vi "DualPump_ExplicitControl_ReverseFlow.vi"() -> ()   [LabVIEW 2025]
uses:
  <vilib>/Utility/error.llb/DialogType.ctl
panel:
  in  "quit":bool
  in  "Tab Control":enum32{"Control Interface", "Info and Help"}(tab)
  out "Pump #2 Sucked Amount (µL)":dbl
  out "Pump #1 Sucked Amount (µL)":dbl
  in  "Pump #2 Start/Stop Button":bool
  in  "Pump #1 COM port":refnum<visa-resource-name>
  in  "Pump #1 flow rate (µL/min)":dbl=2000.0 format="%.3f"
  in  "Pump #2 COM port":refnum<visa-resource-name>
  in  "Pump #2 flow rate (µL/min)":dbl=5000.0 format="%.3f"
  in  "Pump #2 Suck Amount (µL)":dbl=75.0 format="%.3f"
  out "Pump #2 Flowing":bool
  in  "Pump 1 Connect":bool
  in  "Pump 2 Connect":bool
  out "Pump 2 Connected":bool
  out "Pump 1 Connected":bool
  in  "Pump #1 Suck Amount (µL)":dbl=200.0
  in  "Pump #1 Flavor Blast Button":bool
  in  "Pump #1 Start/Stop Button":bool
  out "Pump #1 Flowing":bool
  in  "Pump #2 Flavor Blast Button":bool
  out "Interface Locked":bool
  out "Pump #2 Purging":bool
  in  "Pump #1 Full Purge Button":bool
  in  "Pump #2 Partial Purge Amount (µL)":dbl
  in  "Pump #2 Partial Purge Button":bool
  out "Pump #2 Amount in Syringe (µL)":dbl
  out "Pump #1 Amount in Syringe (µL)":dbl
  in  "Pump #2 syringe volume":dbl(ring)=28.75 items=["5 mL"=11.43, "15 mL"=18.034, "20 mL"=19.79, "50 mL"=28.75]
  in  "Pump #1 syringe volume":dbl(ring)=28.75 items=["5 mL"=11.43, "15 mL"=18.034, "20 mL"=19.79, "50 mL"=28.75, ""=0.0]
  in  "Pump #1 Partial Purge Button":bool
  in  "Pump #2 Full Purge\n Button":bool
  in  "Pump #1 Partial Purge Amount (µL)":dbl
  out "Pump #1 Purging":bool
  # "THIS VI IS FOR DIRECTION-REVERSED FLOW - USE ONLY FOR FILLING SYRINGES AT SET RATES"
  # "1. Set Communication"
  # "Pump #1"
  # "Pump #2"
  # "This program is designed to only control the two New Era Syringe Pumps on-site in the Varro laboratory. It can be generalized for other use by adjusting the hard-coded \"firmware\" variables to match any pump.\n\nFull Purge will empty the syringe completely. Partial Purge will empty the syringe up to the volume injested.\n\nPumps flow continuously when Start is pressed. The pump will suck a specified amount at its flowrate setpoint when Suck It! is pressed.\n\nEmptying and sucking will block the interface, which will be indicated in the upper-right corner."
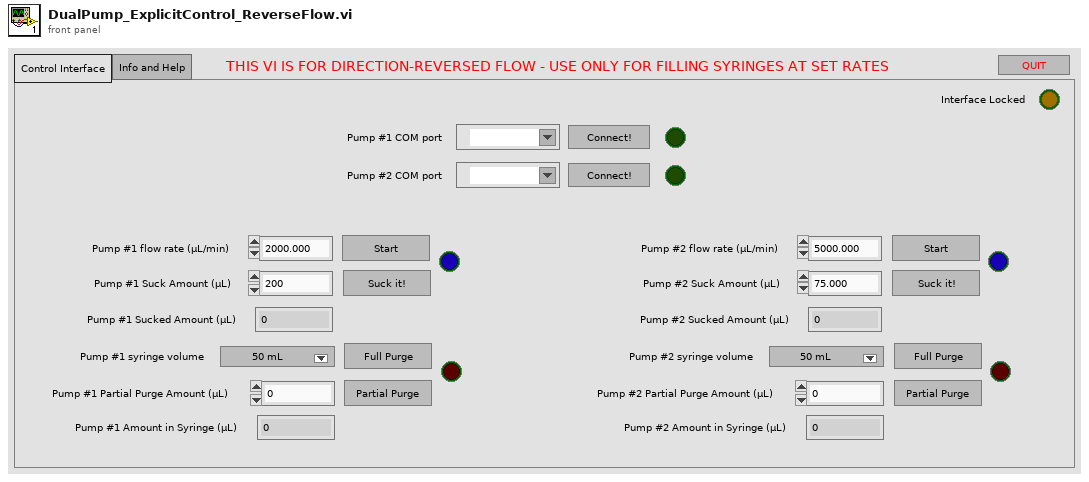
[diagram p1: front panel]
types:
  T1 = cluster{"0=off\n1=on":u16, "Numbers of beeps\n0=continuously":dbl}
  T2 = typedef "DialogType.ctl" = u16
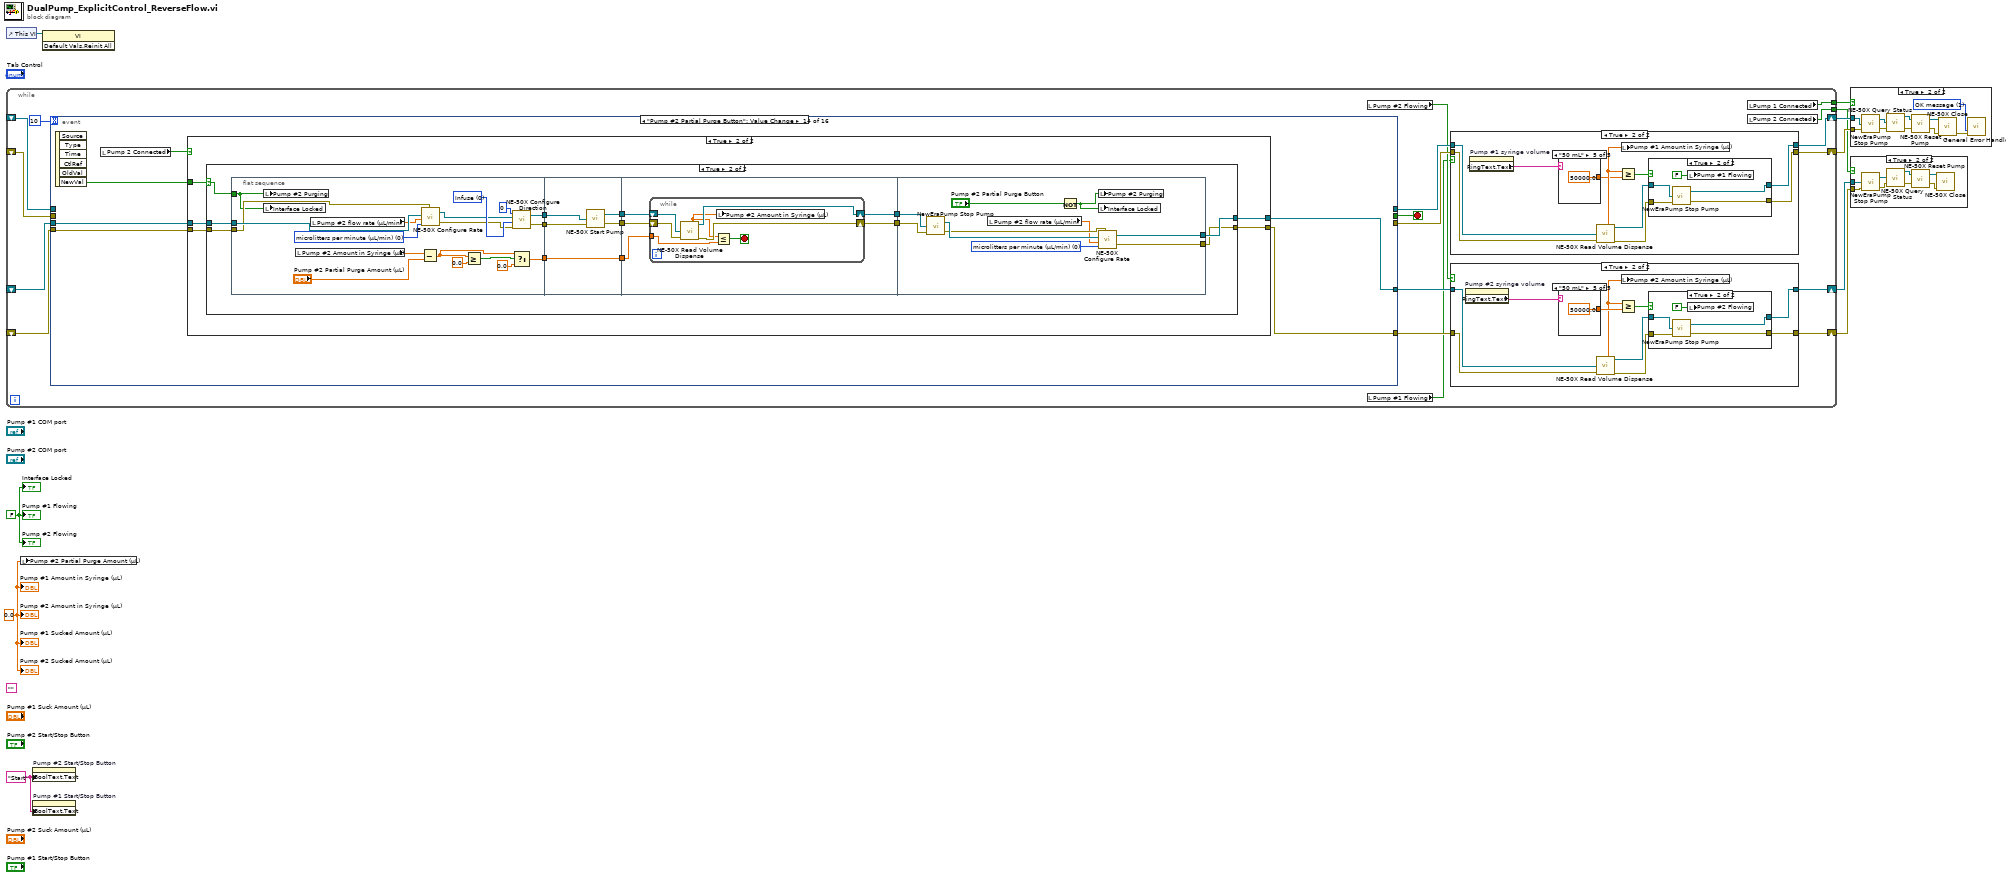
[diagram p0: block diagram]
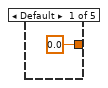
[diagram p6: hidden frame]
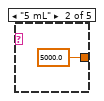
[diagram p7: hidden frame]
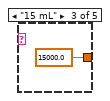
[diagram p8: hidden frame]
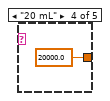
[diagram p9: hidden frame]
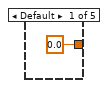
[diagram p12: hidden frame]
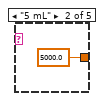
[diagram p13: hidden frame]
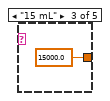
[diagram p14: hidden frame]
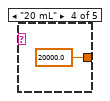
[diagram p15: hidden frame]
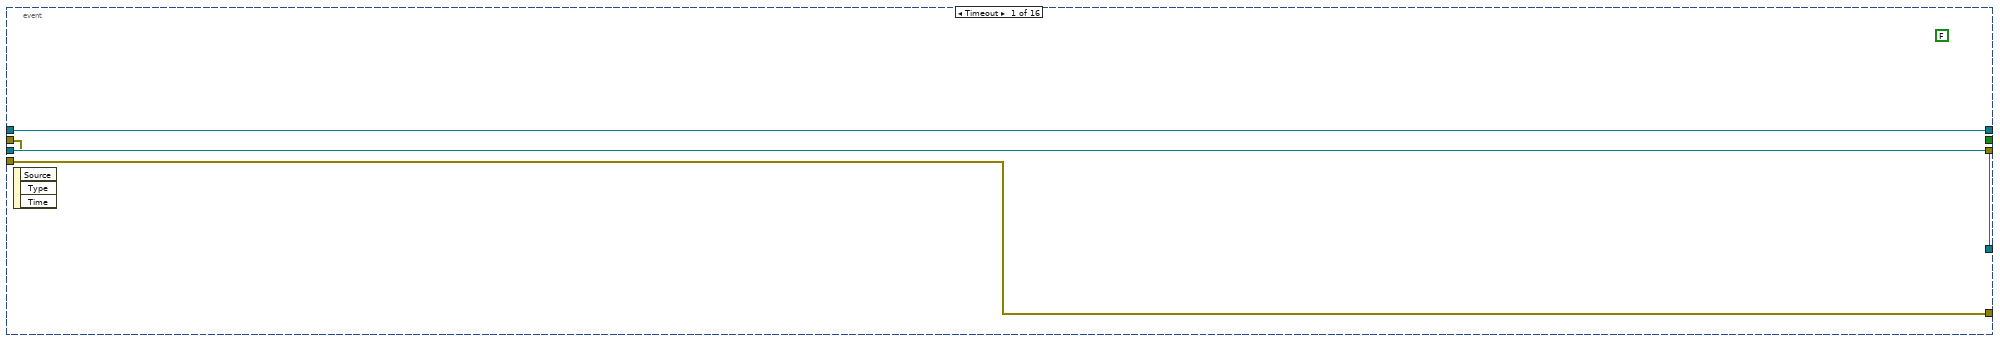
[diagram p16: hidden frame]
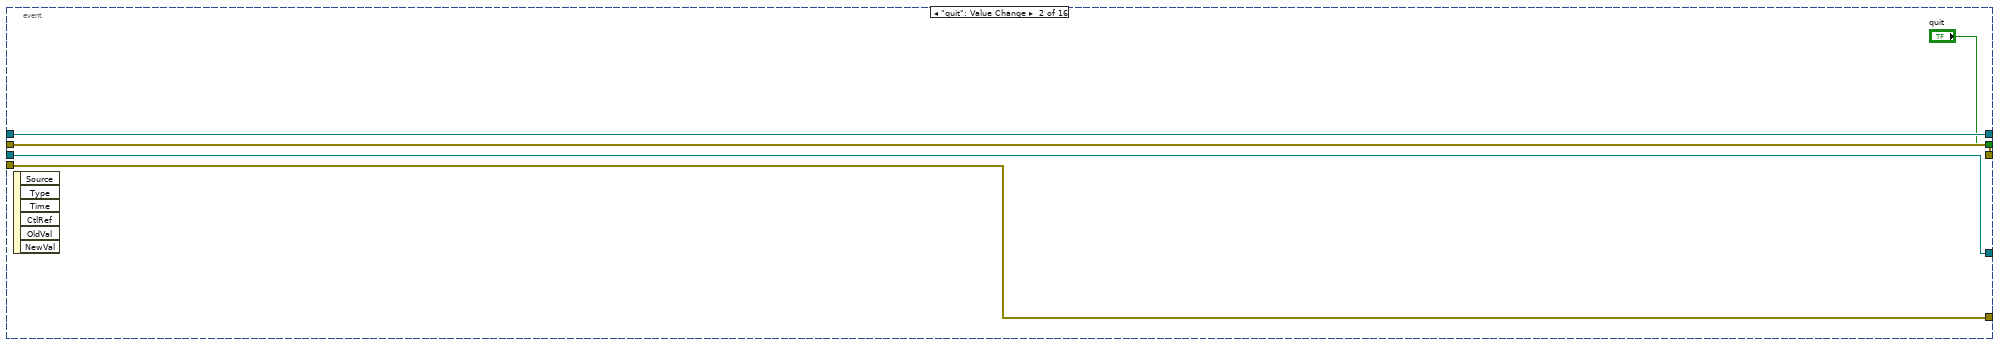
[diagram p17: hidden frame]
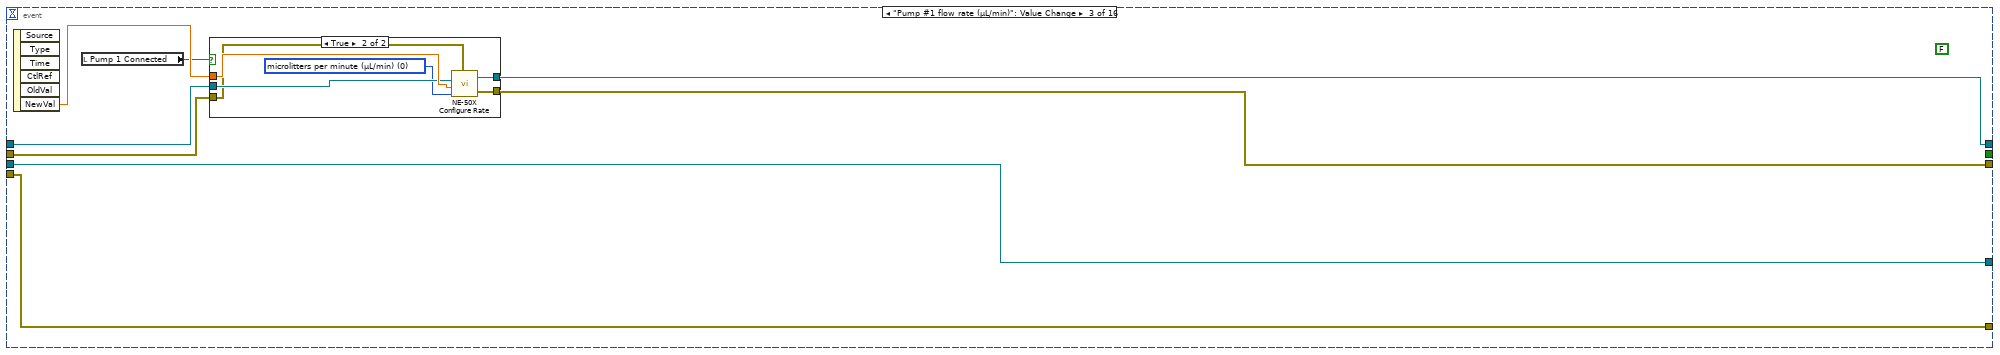
[diagram p18: hidden frame]
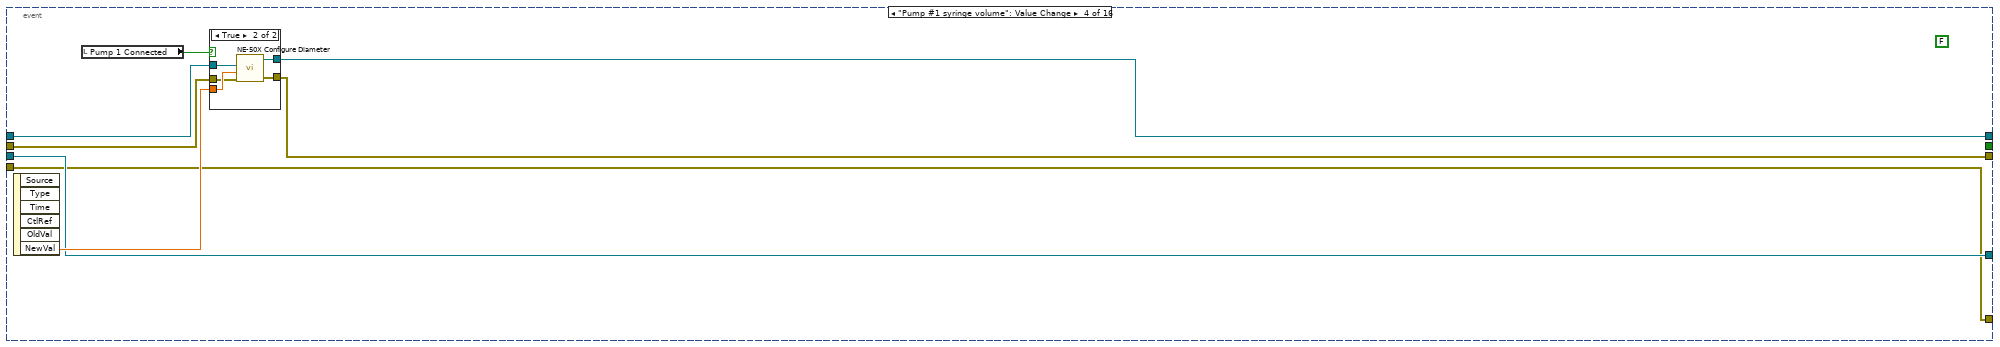
[diagram p20: hidden frame]
diagram:
  w2 = 0.0 ("Pump #1 Flavor Blasted Amount (µL)")
  w1 = FALSE ("0 = Basic")
  w10 = "Start"
  (unwired) ""
  n1 = control-ref of="This VI"() -> (w3:refnum<vi>)
  n2 = while {
    shift-right: [w15] -> w9
    shift-left: _ -> [w28]
    shift-right: [w14] -> w8
    shift-left: _ -> [w27]
    shift-right: [w19] -> w7
    shift-left: _ -> [w25]
    shift-right: [w18] -> w6
    shift-left: _ -> [w26]
    tunnel: [w23] -> w5
    tunnel: [w22] -> w4
    stop <- w11 stop-if-true
    n3 = event shown="[13] \"Pump #2 Partial Purge Button\": Value Change" {
      selector: _ -> [_ _ _ _ _ _ _ _ _ _ _ _ _ _ _ _]
      dyn-events: _ -> [_ _ _ _ _ _ _ _ _ _ _ _ _ _ _ _]
      timeout: 10 -> [_ _ _ _ _ _ _ _ _ _ _ _ _ _ _ _]
      tunnel: w28 -> [w80 w83 w88 w104 w119 w153 w248 w263 w279 w309 w400 _ w476 w555 w629 w706]
      tunnel: w27 -> [w79 w82 w87 w103 w118 w152 w247 w262 w278 w308 w399 _ w475 w554 w628 w705]
      tunnel: w25 -> [w78 w85 w92 w108 w124 w151 w243 w259 w273 w303 _ w439 w481 _ w632 w702]
      tunnel: w26 -> [w77 w84 w91 w107 w122 w150 w242 w258 w272 w301 _ w438 w480 _ w633 w699]
      tunnel: [w80 w83 w88 w104 w119 w147 w246 w261 w275 w307 w400 w441 w476 w553 w629 w701] -> w17
      tunnel: [w79 w82 w87 w103 w118 w148 w245 w260 w274 w306 w399 w440 w475 w552 w628 w700] -> w16
      tunnel: [w78 w85 w90 w106 w123 w146 w243 w259 w273 w304 w403 w439 w478 _ w631 w702] -> w21
      tunnel: [w77 w84 w89 w105 w121 w145 w242 w258 w272 w302 w402 w438 w477 _ w630 w699] -> w20
      tunnel: [_ "quit" _ _ _ _ _ _ _ _ _ _ _ _ _ _] -> w11
      event Timeout {
        (unwired) FALSE ("quit")
        n4 = event-data() -> ()  [unwired: 1 in, 3 out]
      }
      event "quit": Value Change {
        n5 = event-data() -> ()  [unwired: 1 in, 6 out]
      }
      event "Pump #1 flow rate (µL/min)": Value Change {
        (unwired) FALSE ("quit")
        n6 = event-data() -> ("NewVal"=w93:dbl)  [unwired: 1 in, 5 out]
        n7 = local read "Pump 1 Connected"() -> (w86:bool)
        n8 = case shown="True" w86 {
          tunnel: w93 -> [_ w101]
          tunnel: w92 -> [w95 w100]
          tunnel: w91 -> [w94 w99]
          tunnel: [w95 w97] -> w90
          tunnel: [w94 w96] -> w89
          frame False {
          }
          frame True {
            w98 = 0 items=["microlitters per minute (µL/min)", "microlitters per hour (µL/hr)", "milliliters per minute (mL/min)", "milliliters per hour (µL/hr)"] ("Units")
            n9 = call <instrlib>:"NE-50X Configure Rate.vi"("VISA resource name"=w100, "Flow"=w101, "Units"=w98, "error in (no error)"=w99) -> ("VISA resource name out"=w97:refnum<visa-resource-name>, "error out"=w96:errorcluster)  [unwired: 1 in]
          }
        }
      }
      event "Pump #1 syringe volume": Value Change {
        (unwired) FALSE ("quit")
        n10 = event-data() -> ("NewVal"=w109:dbl)  [unwired: 1 in, 5 out]
        n11 = local read "Pump 1 Connected"() -> (w102:bool)
        n12 = case shown="True" w102 {
          tunnel: w109 -> [_ w116]
          tunnel: w108 -> [w110 w115]
          tunnel: w107 -> [w111 w114]
          tunnel: [w110 w113] -> w106
          tunnel: [w111 w112] -> w105
          frame False {
          }
          frame True {
            n13 = call <instrlib>:"NE-50X Configure Diameter.vi"("error in (no error)"=w114, "Diameter (19.58 mm)"=w116, "VISA resource name"=w115) -> ("error out"=w112:errorcluster, "VISA resource name out"=w113:refnum<visa-resource-name>)  [unwired: 1 in, 1 out]
          }
        }
      }
      event "Pump #1 Start/Stop Button": Value Change {
        n14 = event-data() -> ("NewVal"=w120:bool)  [unwired: 1 in, 5 out]
        n15 = local write "Pump #1 Flowing"(w120) -> ()
        n16 = local read "Pump 1 Connected"() -> (w117:bool)
        n17 = case shown="True" w117 {
          tunnel: w124 -> [w126 w131]
          tunnel: [w126 w134] -> w123
          tunnel: w122 -> [w125 w130]
          tunnel: [w125 w133] -> w121
          tunnel: w120 -> [_ w132]
          frame False {
          }
          frame True {
            w129 = u16 1 items=["Infuse", "Withdraw"] ("Direction")
            n18 = call <instrlib>:"NE-50X Configure Direction.vi"("error in (no error)"=w130, "Direction"=w129, "VISA resource name"=w131) -> ("error out"=w127:errorcluster, "VISA resource name out"=w128:refnum<visa-resource-name>)  [unwired: 1 in]
            n19 = case shown="False" w132 {
              tunnel: [w139 w143] -> w134
              tunnel: [w138 w142] -> w133
              tunnel: w128 -> [w136 w141]
              tunnel: w127 -> [w135 w140]
              frame False {
                n20 = call <instrlib>:"NewEraPump Stop Pump.vi"("error in (no error)"=w135, "VISA resource name"=w136) -> ("error out"=w138:errorcluster, "VISA resource name out"=w139:refnum<visa-resource-name>)  [unwired: 1 in]
                n21 = property on="Pump #1 Start/Stop Button" class="Bool"("BoolText.Text"="Start" ("Boolean Text.Text")) -> ()  [unwired: 2 in, 2 out]
              }
              frame True {
                n22 = call <instrlib>:"NE-50X Start Pump.vi"("error in (no error)"=w140, "VISA resource name"=w141) -> ("error out"=w142:errorcluster, "VISA resource name out"=w143:refnum<visa-resource-name>)  [unwired: 1 in]
                n23 = property on="Pump #1 Start/Stop Button" class="Bool"("BoolText.Text"="Stop" ("Boolean Text.Text")) -> ()  [unwired: 2 in, 2 out]
              }
            }
          }
        }
      }
      event "Pump #1 Flavor Blast Button": Value Change {
        (unwired) FALSE ("quit")
        n24 = event-data() -> ("NewVal"=w149:bool)  [unwired: 1 in, 5 out]
        n25 = local read "Pump 1 Connected"() -> (w154:bool)
        n26 = case shown="True" w154 {
          tunnel: w151 -> [w156 w167]
          tunnel: w150 -> [w155 w166]
          tunnel: [w156 w165] -> w146
          tunnel: [w155 w164] -> w145
          tunnel: w149 -> [_ w163]
          tunnel: [w158 w162] -> w147
          tunnel: w153 -> [w158 w161]
          tunnel: [w157 w160] -> w148
          tunnel: w152 -> [w157 w159]
          frame False {
          }
          frame True {
            n27 = case shown="True" w163 {
              selector: w163 -> [_ w174]
              tunnel: w167 -> [w173 w196]
              tunnel: [w171 w190] -> w165
              tunnel: w166 -> [w172 w195]
              tunnel: [w170 w189] -> w164
              tunnel: [w169 w188] -> w162
              tunnel: w161 -> [w169 w185]
              tunnel: [w168 w184] -> w160
              tunnel: w159 -> [w168 w181]
              frame False {
                n28 = call <instrlib>:"NewEraPump Stop Pump.vi"("error in (no error)"=w172, "VISA resource name"=w173) -> ("error out"=w170:errorcluster, "VISA resource name out"=w171:refnum<visa-resource-name>)  [unwired: 1 in]
              }
              frame True {
                n29 = flat-sequence {
                  tunnel: [w200] -> w180
                  tunnel: [w199] -> w179
                  tunnel: [w208] -> w178
                  tunnel: [w207] -> w177
                  tunnel: [w197] -> w175
                  tunnel: w196 -> [w206]
                  tunnel: w195 -> [w205]
                  tunnel: w185 -> [w208]
                  tunnel: w181 -> [w207]
                  tunnel: w174 -> [w198]
                  tunnel: w180 -> [w216]
                  tunnel: w179 -> [w215]
                  tunnel: [w214] -> w194
                  tunnel: [w213] -> w193
                  tunnel: [w212] -> w186
                  tunnel: w178 -> [w212]
                  tunnel: [w211] -> w182
                  tunnel: w177 -> [w211]
                  tunnel: [w210] -> w176
                  tunnel: w175 -> [w210]
                  tunnel: w194 -> [w223]
                  tunnel: w193 -> [w222]
                  tunnel: [w221] -> w192
                  tunnel: [w220] -> w191
                  tunnel: [w219] -> w187
                  tunnel: w186 -> [w219]
                  tunnel: [w218] -> w183
                  tunnel: w182 -> [w218]
                  tunnel: w176 -> [w217]
                  tunnel: w192 -> [w240]
                  tunnel: w191 -> [w239]
                  tunnel: [w238] -> w190
                  tunnel: [w237] -> w189
                  tunnel: [w236] -> w188
                  tunnel: w187 -> [w236]
                  tunnel: [w235] -> w184
                  tunnel: w183 -> [w235]
                  frame #0 {
                    w204 = u16 1 items=["Infuse", "Withdraw"] ("Direction")
                    n30 = local write "Interface Locked"(w198) -> ()
                    n31 = local write "Pump #1 Sucked Amount (µL)"(0.0 ("Pump #1 Flavor Blasted Amount (µL)")) -> ()
                    n32 = call <instrlib>:"NE-50X Configure Direction.vi"("error in (no error)"=w205, "Direction"=w204, "VISA resource name"=w206) -> ("error out"=w202:errorcluster, "VISA resource name out"=w201:refnum<visa-resource-name>)  [unwired: 1 in]
                    n33 = call <instrlib>:"NE-50X Read Volume Dispense.vi"("VISA resource name"=w201, "error in (no error)"=w202) -> ("VISA resource name out"=w200:refnum<visa-resource-name>, "Withdrawn Volume (uL)"=w197:dbl, "error out"=w199:errorcluster)  [unwired: 1 in, 2 out]
                  }
                  frame #1 {
                    n34 = call <instrlib>:"NE-50X Start Pump.vi"("error in (no error)"=w215, "VISA resource name"=w216) -> ("error out"=w213:errorcluster, "VISA resource name out"=w214:refnum<visa-resource-name>)  [unwired: 1 in]
                    n35 = local write "Pump #1 Flowing"(TRUE) -> ()
                  }
                  frame #2 {
                    n36 = while {
                      shift-right: [w230] -> w221
                      shift-left: w223 -> [w233]
                      shift-right: [w229] -> w220
                      shift-left: w222 -> [w232]
                      tunnel: w217 -> [w227]
                      stop <- w231 stop-if-true
                      n37 = call <instrlib>:"NE-50X Read Volume Dispense.vi"("VISA resource name"=w233, "error in (no error)"=w232) -> ("VISA resource name out"=w230:refnum<visa-resource-name>, "Withdrawn Volume (uL)"=w224:dbl, "error out"=w229:errorcluster, "Amount Remaining (uL)"=w225:dbl)  [unwired: 1 in, 1 out]
                      n38 = local read "Pump #1 Suck Amount (µL)"() -> (w228:dbl)
                      n39 = Subtract(x=w224, y=w227) -> (x-y=w226:dbl)
                      n40 = local write "Pump #1 Amount in Syringe (µL)"(w225) -> ()
                      n41 = local write "Pump #1 Sucked Amount (µL)"(w226) -> ()
                      n42 = Greater Or Equal?(x=w226, y=w228) -> (x >= y?=w231:bool)
                    }
                  }
                  frame #3 {
                    w234 = FALSE
                    n43 = call <instrlib>:"NewEraPump Stop Pump.vi"("error in (no error)"=w239, "VISA resource name"=w240) -> ("error out"=w237:errorcluster, "VISA resource name out"=w238:refnum<visa-resource-name>)  [unwired: 1 in]
                    n44 = local write "Pump #1 Flowing"(w234) -> ()
                    n45 = local write "Interface Locked"(w234) -> ()
                  }
                }
              }
            }
          }
        }
      }
      event "Pump #2 flow rate (µL/min)": Value Change {
        (unwired) FALSE ("quit")
        n46 = event-data() -> ("NewVal"=w244:dbl)  [unwired: 1 in, 5 out]
        n47 = local read "Pump 2 Connected"() -> (w241:bool)
        n48 = case shown="True" w241 {
          tunnel: w248 -> [w250 w256]
          tunnel: w247 -> [w249 w255]
          tunnel: [w250 w254] -> w246
          tunnel: [w249 w253] -> w245
          tunnel: w244 -> [_ w252]
          frame False {
          }
          frame True {
            w251 = 0 items=["microlitters per minute (µL/min)", "microlitters per hour (µL/hr)", "milliliters per minute (mL/min)", "milliliters per hour (µL/hr)"] ("Units")
            n49 = call <instrlib>:"NE-50X Configure Rate.vi"("VISA resource name"=w256, "Flow"=w252, "Units"=w251, "error in (no error)"=w255) -> ("VISA resource name out"=w254:refnum<visa-resource-name>, "error out"=w253:errorcluster)  [unwired: 1 in]
          }
        }
      }
      event "Pump #2 syringe volume": Value Change {
        (unwired) FALSE ("quit")
        n50 = event-data() -> ("NewVal"=w264:dbl)  [unwired: 1 in, 5 out]
        n51 = local read "Pump 2 Connected"() -> (w257:bool)
        n52 = case shown="True" w257 {
          tunnel: w264 -> [_ w271]
          tunnel: w263 -> [w265 w270]
          tunnel: w262 -> [w266 w269]
          tunnel: [w265 w268] -> w261
          tunnel: [w266 w267] -> w260
          frame False {
          }
          frame True {
            n53 = call <instrlib>:"NE-50X Configure Diameter.vi"("error in (no error)"=w269, "Diameter (19.58 mm)"=w271, "VISA resource name"=w270) -> ("error out"=w267:errorcluster, "VISA resource name out"=w268:refnum<visa-resource-name>)  [unwired: 1 in, 1 out]
          }
        }
      }
      event "Pump #2 Start/Stop Button": Value Change {
        n54 = event-data() -> ("NewVal"=w276:bool)  [unwired: 1 in, 5 out]
        n55 = local write "Pump #2 Flowing"(w276) -> ()
        n56 = local read "Pump 2 Connected"() -> (w277:bool)
        n57 = case shown="True" w277 {
          tunnel: w279 -> [w281 w286]
          tunnel: [w281 w289] -> w275
          tunnel: w278 -> [w280 w284]
          tunnel: [w280 w288] -> w274
          tunnel: w276 -> [_ w287]
          frame False {
          }
          frame True {
            w282 = u16 1 items=["Infuse", "Withdraw"] ("Direction")
            n58 = call <instrlib>:"NE-50X Configure Direction.vi"("error in (no error)"=w284, "Direction"=w282, "VISA resource name"=w286) -> ("error out"=w283:errorcluster, "VISA resource name out"=w285:refnum<visa-resource-name>)  [unwired: 1 in]
            n59 = case shown="False" w287 {
              tunnel: w285 -> [w294 w298]
              tunnel: [w292 w297] -> w289
              tunnel: w283 -> [w293 w296]
              tunnel: [w291 w295] -> w288
              frame False {
                n60 = call <instrlib>:"NewEraPump Stop Pump.vi"("error in (no error)"=w293, "VISA resource name"=w294) -> ("error out"=w291:errorcluster, "VISA resource name out"=w292:refnum<visa-resource-name>)  [unwired: 1 in]
                n61 = property on="Pump #2 Start/Stop Button" class="Bool"("BoolText.Text"="Start" ("Boolean Text.Text")) -> ()  [unwired: 2 in, 2 out]
              }
              frame True {
                n62 = call <instrlib>:"NE-50X Start Pump.vi"("error in (no error)"=w296, "VISA resource name"=w298) -> ("error out"=w295:errorcluster, "VISA resource name out"=w297:refnum<visa-resource-name>)  [unwired: 1 in]
                n63 = property on="Pump #2 Start/Stop Button" class="Bool"("BoolText.Text"="Stop" ("Boolean Text.Text")) -> ()  [unwired: 2 in, 2 out]
              }
            }
          }
        }
      }
      event "Pump #2 Flavor Blast Button": Value Change {
        (unwired) FALSE ("quit")
        n64 = event-data() -> ("NewVal"=w305:bool)  [unwired: 1 in, 5 out]
        n65 = local read "Pump 2 Connected"() -> (w300:bool)
        n66 = case shown="True" w300 {
          tunnel: w309 -> [w311 w322]
          tunnel: w308 -> [w310 w321]
          tunnel: [w311 w320] -> w307
          tunnel: [w310 w319] -> w306
          tunnel: w305 -> [_ w318]
          tunnel: [w313 w317] -> w304
          tunnel: w303 -> [w313 w316]
          tunnel: [w312 w315] -> w302
          tunnel: w301 -> [w312 w314]
          frame False {
          }
          frame True {
            n67 = case shown="True" w318 {
              selector: w318 -> [_ w330]
              tunnel: w322 -> [w329 w352]
              tunnel: [w327 w346] -> w320
              tunnel: w321 -> [w328 w351]
              tunnel: [w326 w345] -> w319
              tunnel: [w324 w344] -> w317
              tunnel: w316 -> [w324 w341]
              tunnel: [w323 w340] -> w315
              tunnel: w314 -> [w323 w337]
              frame False {
                n68 = property on="Pump #2 Flowing" class="Bool (strict)"("BoolText.Text"="Start" ("Boolean Text.Text")) -> ()  [unwired: 2 in, 2 out]
                n69 = call <instrlib>:"NewEraPump Stop Pump.vi"("error in (no error)"=w328, "VISA resource name"=w329) -> ("error out"=w326:errorcluster, "VISA resource name out"=w327:refnum<visa-resource-name>)  [unwired: 1 in]
              }
              frame True {
                n70 = flat-sequence {
                  tunnel: [w364] -> w336
                  tunnel: [w363] -> w335
                  tunnel: w352 -> [w361]
                  tunnel: w351 -> [w362]
                  tunnel: w341 -> [w364]
                  tunnel: w337 -> [w363]
                  tunnel: [w357] -> w334
                  tunnel: [w356] -> w333
                  tunnel: [w353] -> w331
                  tunnel: w330 -> [w354]
                  tunnel: [w370] -> w350
                  tunnel: [w369] -> w349
                  tunnel: [w368] -> w342
                  tunnel: w336 -> [w368]
                  tunnel: [w367] -> w338
                  tunnel: w335 -> [w367]
                  tunnel: w334 -> [w372]
                  tunnel: w333 -> [w371]
                  tunnel: [w366] -> w332
                  tunnel: w331 -> [w366]
                  tunnel: w350 -> [w379]
                  tunnel: w349 -> [w378]
                  tunnel: [w377] -> w348
                  tunnel: [w376] -> w347
                  tunnel: [w375] -> w343
                  tunnel: w342 -> [w375]
                  tunnel: [w374] -> w339
                  tunnel: w338 -> [w374]
                  tunnel: w332 -> [w373]
                  tunnel: w348 -> [w396]
                  tunnel: w347 -> [w395]
                  tunnel: [w394] -> w346
                  tunnel: [w393] -> w345
                  tunnel: [w392] -> w344
                  tunnel: w343 -> [w392]
                  tunnel: [w391] -> w340
                  tunnel: w339 -> [w391]
                  frame #0 {
                    w360 = u16 1 items=["Infuse", "Withdraw"] ("Direction")
                    n71 = local write "Interface Locked"(w354) -> ()
                    n72 = local write "Pump #2 Sucked Amount (µL)"(0.0 ("Pump #2 Flavor Blasted Amount (µL)")) -> ()
                    n73 = call <instrlib>:"NE-50X Configure Direction.vi"("error in (no error)"=w362, "Direction"=w360, "VISA resource name"=w361) -> ("error out"=w358:errorcluster, "VISA resource name out"=w359:refnum<visa-resource-name>)  [unwired: 1 in]
                    n74 = call <instrlib>:"NE-50X Read Volume Dispense.vi"("VISA resource name"=w359, "error in (no error)"=w358) -> ("VISA resource name out"=w357:refnum<visa-resource-name>, "Withdrawn Volume (uL)"=w353:dbl, "error out"=w356:errorcluster)  [unwired: 1 in, 2 out]
                  }
                  frame #1 {
                    n75 = call <instrlib>:"NE-50X Start Pump.vi"("error in (no error)"=w371, "VISA resource name"=w372) -> ("error out"=w369:errorcluster, "VISA resource name out"=w370:refnum<visa-resource-name>)  [unwired: 1 in]
                    n76 = local write "Pump #2 Flowing"(TRUE) -> ()
                  }
                  frame #2 {
                    n77 = while {
                      shift-right: [w385] -> w377
                      shift-left: w379 -> [w389]
                      shift-right: [w384] -> w376
                      shift-left: w378 -> [w388]
                      tunnel: w373 -> [w383]
                      stop <- w387 stop-if-true
                      n78 = call <instrlib>:"NE-50X Read Volume Dispense.vi"("VISA resource name"=w389, "error in (no error)"=w388) -> ("VISA resource name out"=w385:refnum<visa-resource-name>, "Withdrawn Volume (uL)"=w380:dbl, "error out"=w384:errorcluster, "Amount Remaining (uL)"=w381:dbl)  [unwired: 1 in, 1 out]
                      n79 = local read "Pump #2 Suck Amount (µL)"() -> (w386:dbl)
                      n80 = Subtract(x=w380, y=w383) -> (x-y=w382:dbl)
                      n81 = local write "Pump #2 Amount in Syringe (µL)"(w381) -> ()
                      n82 = local write "Pump #2 Sucked Amount (µL)"(w382) -> ()
                      n83 = Greater Or Equal?(x=w382, y=w386) -> (x >= y?=w387:bool)
                    }
                  }
                  frame #3 {
                    w390 = FALSE
                    n84 = call <instrlib>:"NewEraPump Stop Pump.vi"("error in (no error)"=w395, "VISA resource name"=w396) -> ("error out"=w393:errorcluster, "VISA resource name out"=w394:refnum<visa-resource-name>)  [unwired: 1 in]
                    n85 = local write "Pump #2 Flowing"(w390) -> ()
                    n86 = local write "Interface Locked"(w390) -> ()
                  }
                }
              }
            }
          }
        }
      }
      event "Pump 1 Connect": Value Change {
        w406 = 0 items=["microlitters per minute (µL/min)", "microlitters per hour (µL/hr)", "milliliters per minute (mL/min)", "milliliters per hour (µL/hr)"] ("Units")
        w397 = u16 1 items=["Infuse", "Withdraw"] ("Direction")
        w411 = 0
        w404 = u16 0 items=["Off", "On"] ("0 = Disabled")
        n87 = event-data() -> ()  [unwired: 1 in, 6 out]
        n88 = local read "Pump #1 COM port"() -> (w401:refnum<visa-resource-name>)
        n89 = call <instrlib>:"NE-50X Initialize.vi"("Baud Rate (19200)"=19200, "VISA resource name"=w401) -> ("error out"=w414:errorcluster, "VISA resource name out"=w433:refnum<visa-resource-name>)  [unwired: 1 in]
        n90 = call <instrlib>:"NE-50X Read Firmware Version.vi"("error in (no error)"=w414, "VISA resource name"=w433, "Address (0 if unused)"=w411) -> ("error out"=w415:errorcluster, "Version"=w434:string, "VISA resource name out"=w432:refnum<visa-resource-name>)
        n91 = Equal?(x="NE1000V3.934", y=w434) -> (x = y?=→"Pump 1 Connected":bool)
        n92 = call <instrlib>:"NE-50X Configure Alarms.vi"("error in (no error)"=w415, "Audible Alarms"=FALSE, "VISA resource name"=w432, "Address (0)"=w411) -> ("error out"=w416:errorcluster, "VISA resource name out"=w431:refnum<visa-resource-name>)
        n93 = call <instrlib>:"NE-50X Configure Power Failure Mode.vi"("error in (no error)"=w416, "Power Failure Mode"=w404, "VISA resource name"=w431, "Address (0)"=w411) -> ("error out"=w417:errorcluster, "VISA resource name out"=w430:refnum<visa-resource-name>)
        n94 = call <instrlib>:"NE-50X Configure Safe Mode.vi"("error in (no error)"=w417, "Safe Mode"=FALSE ("0 = Basic"), "VISA resource name"=w430, "Address (0)"=w411) -> ("error out"=w421:errorcluster, "VISA resource name out"=w429:refnum<visa-resource-name>)
        n95 = call <instrlib>:"NE-50X Clear Volumes.vi"("error in (no error)"=w421, "VISA resource name"=w429, "Address (0)"=w411) -> ("error out"=w413:errorcluster, "VISA resource name out"=w428:refnum<visa-resource-name>)
        n96 = call <instrlib>:"NE-50X Configure Diameter.vi"("error in (no error)"=w413, "Diameter (19.58 mm)"="Pump #1 syringe volume", "VISA resource name"=w428, "Address (0)"=w411) -> ("error out"=w422:errorcluster, "VISA resource name out"=w427:refnum<visa-resource-name>)  [unwired: 1 out]
        n97 = call <instrlib>:"NE-50X Configure Rate.vi"("Address (0)"=w411, "VISA resource name"=w427, "Flow"="Pump #1 flow rate (µL/min)", "Units"=w406, "error in (no error)"=w422) -> ("VISA resource name out"=w426:refnum<visa-resource-name>, "error out"=w420:errorcluster)
        n98 = call <instrlib>:"NE-50X Configure Volume.vi"("error in (no error)"=w420, "Volume"=0.0, "VISA resource name"=w426, "Address (0)"=w411) -> ("error out"=w419:errorcluster, "VISA resource name out"=w425:refnum<visa-resource-name>)
        n99 = call <instrlib>:"NE-50X Configure Direction.vi"("error in (no error)"=w419, "Direction"=w397, "VISA resource name"=w425, "Address (0)"=w411) -> ("error out"=w418:errorcluster, "VISA resource name out"=w424:refnum<visa-resource-name>)
        n100 = call <instrlib>:"NE-50X Buzzer.vi"("error in (no error)"=w418, "Buzzer"=T1 {"0=off\n1=on"=0, "Numbers of beeps\n0=continuously"=1.0}, "VISA resource name"=w424, "Address (0)"=w411) -> ("error out"=w402:errorcluster, "VISA resource name out"=w403:refnum<visa-resource-name>)
      }
      event "Pump 2 Connect": Value Change {
        (unwired) FALSE ("quit")
        w448 = 0
        w446 = 0 items=["microlitters per minute (µL/min)", "microlitters per hour (µL/hr)", "milliliters per minute (mL/min)", "milliliters per hour (µL/hr)"] ("Units")
        w436 = u16 1 items=["Infuse", "Withdraw"] ("Direction")
        w444 = u16 0 items=["Off", "On"] ("0 = Disabled")
        n101 = event-data() -> ()  [unwired: 1 in, 6 out]
        n102 = local read "Pump #2 COM port"() -> (w451:refnum<visa-resource-name>)
        n103 = call <instrlib>:"NE-50X Initialize.vi"("Baud Rate (19200)"=19200, "VISA resource name"=w451) -> ("error out"=w453:errorcluster, "VISA resource name out"=w472:refnum<visa-resource-name>)  [unwired: 1 in]
        n104 = call <instrlib>:"NE-50X Read Firmware Version.vi"("error in (no error)"=w453, "VISA resource name"=w472, "Address (0 if unused)"=w448) -> ("error out"=w454:errorcluster, "Version"=w473:string, "VISA resource name out"=w471:refnum<visa-resource-name>)
        n105 = Equal?(x="NE1010V3.934", y=w473) -> (x = y?=→"Pump 2 Connected":bool)
        n106 = call <instrlib>:"NE-50X Configure Alarms.vi"("error in (no error)"=w454, "Audible Alarms"=FALSE, "VISA resource name"=w471, "Address (0)"=w448) -> ("error out"=w455:errorcluster, "VISA resource name out"=w470:refnum<visa-resource-name>)
        n107 = call <instrlib>:"NE-50X Configure Power Failure Mode.vi"("error in (no error)"=w455, "Power Failure Mode"=w444, "VISA resource name"=w470, "Address (0)"=w448) -> ("error out"=w456:errorcluster, "VISA resource name out"=w469:refnum<visa-resource-name>)
        n108 = call <instrlib>:"NE-50X Configure Safe Mode.vi"("error in (no error)"=w456, "Safe Mode"=FALSE ("0 = Basic"), "VISA resource name"=w469, "Address (0)"=w448) -> ("error out"=w460:errorcluster, "VISA resource name out"=w468:refnum<visa-resource-name>)
        n109 = call <instrlib>:"NE-50X Clear Volumes.vi"("error in (no error)"=w460, "VISA resource name"=w468, "Address (0)"=w448) -> ("error out"=w452:errorcluster, "VISA resource name out"=w467:refnum<visa-resource-name>)
        n110 = call <instrlib>:"NE-50X Configure Diameter.vi"("error in (no error)"=w452, "Diameter (19.58 mm)"="Pump #2 syringe volume", "VISA resource name"=w467, "Address (0)"=w448) -> ("error out"=w461:errorcluster, "VISA resource name out"=w466:refnum<visa-resource-name>)  [unwired: 1 out]
        n111 = call <instrlib>:"NE-50X Configure Rate.vi"("Address (0)"=w448, "VISA resource name"=w466, "Flow"="Pump #2 flow rate (µL/min)", "Units"=w446, "error in (no error)"=w461) -> ("VISA resource name out"=w465:refnum<visa-resource-name>, "error out"=w459:errorcluster)
        n112 = call <instrlib>:"NE-50X Configure Volume.vi"("error in (no error)"=w459, "Volume"=0.0, "VISA resource name"=w465, "Address (0)"=w448) -> ("error out"=w458:errorcluster, "VISA resource name out"=w464:refnum<visa-resource-name>)
        n113 = call <instrlib>:"NE-50X Configure Direction.vi"("error in (no error)"=w458, "Direction"=w436, "VISA resource name"=w464, "Address (0)"=w448) -> ("error out"=w457:errorcluster, "VISA resource name out"=w463:refnum<visa-resource-name>)
        n114 = call <instrlib>:"NE-50X Buzzer.vi"("error in (no error)"=w457, "Buzzer"=T1 {"0=off\n1=on"=0, "Numbers of beeps\n0=continuously"=1.0}, "VISA resource name"=w463, "Address (0)"=w448) -> ("error out"=w440:errorcluster, "VISA resource name out"=w441:refnum<visa-resource-name>)
      }
      event "Pump #1 Partial Purge Button": Value Change {
        n115 = event-data() -> ("NewVal"=w479:bool)  [unwired: 1 in, 5 out]
        n116 = local read "Pump 1 Connected"() -> (w482:bool)
        n117 = case shown="True" w482 {
          tunnel: [w484 w489] -> w478
          tunnel: [w483 w488] -> w477
          tunnel: w480 -> [w483 w487]
          tunnel: w481 -> [w484 w486]
          tunnel: w479 -> [_ w485]
          frame False {
          }
          frame True {
            n118 = case shown="True" w485 {
              selector: w485 -> [_ w494]
              tunnel: [w493 w502] -> w489
              tunnel: [w492 w501] -> w488
              tunnel: w487 -> [w490 w498]
              tunnel: w486 -> [w491 w497]
              frame False {
                n119 = call <instrlib>:"NewEraPump Stop Pump.vi"("error in (no error)"=w490, "VISA resource name"=w491) -> ("error out"=w492:errorcluster, "VISA resource name out"=w493:refnum<visa-resource-name>)  [unwired: 1 in]
              }
              frame True {
                n120 = flat-sequence {
                  tunnel: [w524] -> w500
                  tunnel: [w523] -> w499
                  tunnel: [w514] -> w495
                  tunnel: w497 -> [w520]
                  tunnel: w498 -> [w518]
                  tunnel: w494 -> [w513]
                  tunnel: w500 -> [w529]
                  tunnel: w499 -> [w528]
                  tunnel: [w527] -> w506
                  tunnel: [w526] -> w505
                  tunnel: [w525] -> w496
                  tunnel: w495 -> [w525]
                  tunnel: w506 -> [w534]
                  tunnel: w505 -> [w533]
                  tunnel: [w532] -> w504
                  tunnel: [w531] -> w503
                  tunnel: w496 -> [w530]
                  tunnel: w504 -> [w548]
                  tunnel: w503 -> [w547]
                  tunnel: [w549] -> w502
                  tunnel: [w551] -> w501
                  frame #0 {
                    w516 = 0 items=["microlitters per minute (µL/min)", "microlitters per hour (µL/hr)", "milliliters per minute (mL/min)", "milliliters per hour (µL/hr)"] ("Units")
                    w522 = u16 0 items=["Infuse", "Withdraw"] ("Direction")
                    n121 = local write "Pump #1 Purging"(w513) -> ()
                    n122 = local write "Interface Locked"(w513) -> ()
                    n123 = local read "Pump #1 Amount in Syringe (µL)"() -> (w510:dbl)
                    n124 = local read "Pump #1 flow rate (µL/min)"() -> (w512:dbl)
                    n125 = Subtract(x=w510, y="Pump #1 Partial Purge Amount (µL)") -> (x-y=w507:dbl)
                    n126 = call <instrlib>:"NE-50X Configure Rate.vi"("VISA resource name"=w520, "Flow"=w512, "Units"=w516, "error in (no error)"=w518) -> ("VISA resource name out"=w519:refnum<visa-resource-name>, "error out"=w517:errorcluster)  [unwired: 1 in]
                    n127 = Greater Or Equal?(x=w507, y=0.0) -> (x >= y?=w515:bool)
                    n128 = call <instrlib>:"NE-50X Configure Direction.vi"("error in (no error)"=w517, "Direction"=w522, "VISA resource name"=w519, "Address (0)"=0) -> ("error out"=w523:errorcluster, "VISA resource name out"=w524:refnum<visa-resource-name>)
                    n129 = Select(t=w507, s=w515, f=0.0) -> (s? t:f=w514:dbl)
                  }
                  frame #1 {
                    n130 = call <instrlib>:"NE-50X Start Pump.vi"("error in (no error)"=w528, "VISA resource name"=w529) -> ("error out"=w526:errorcluster, "VISA resource name out"=w527:refnum<visa-resource-name>)  [unwired: 1 in]
                  }
                  frame #2 {
                    n131 = while {
                      shift-right: [w539] -> w532
                      shift-left: w534 -> [w541]
                      shift-right: [w538] -> w531
                      shift-left: w533 -> [w540]
                      tunnel: w530 -> [w536]
                      stop <- w537 stop-if-true
                      n132 = call <instrlib>:"NE-50X Read Volume Dispense.vi"("VISA resource name"=w541, "error in (no error)"=w540) -> ("VISA resource name out"=w539:refnum<visa-resource-name>, "error out"=w538:errorcluster, "Amount Remaining (uL)"=w535:dbl)  [unwired: 1 in, 2 out]
                      n133 = Less Or Equal?(x=w535, y=w536) -> (x <= y?=w537:bool)
                      n134 = local write "Pump #1 Amount in Syringe (µL)"(w535) -> ()
                    }
                  }
                  frame #3 {
                    w550 = 0 items=["microlitters per minute (µL/min)", "microlitters per hour (µL/hr)", "milliliters per minute (mL/min)", "milliliters per hour (µL/hr)"] ("Units")
                    n135 = call <instrlib>:"NewEraPump Stop Pump.vi"("error in (no error)"=w547, "VISA resource name"=w548) -> ("error out"=w545:errorcluster, "VISA resource name out"=w546:refnum<visa-resource-name>)  [unwired: 1 in]
                    n136 = local read "Pump #1 flow rate (µL/min)"() -> (w544:dbl)
                    n137 = Not(x="Pump #1 Partial Purge Button") -> (.not. x?=w542:bool)
                    n138 = local write "Pump #1 Purging"(w542) -> ()
                    n139 = local write "Interface Locked"(w542) -> ()
                    n140 = call <instrlib>:"NE-50X Configure Rate.vi"("VISA resource name"=w546, "Flow"=w544, "Units"=w550, "error in (no error)"=w545) -> ("VISA resource name out"=w549:refnum<visa-resource-name>, "error out"=w551:errorcluster)  [unwired: 1 in]
                  }
                }
              }
            }
          }
        }
      }
      event "Pump #2 Partial Purge Button": Value Change {
        n141 = event-data() -> ("NewVal"=w556:bool)  [unwired: 1 in, 5 out]
        n142 = local read "Pump 2 Connected"() -> (w557:bool)
        n143 = case shown="True" w557 {
          tunnel: [w559 w564] -> w553
          tunnel: [w558 w563] -> w552
          tunnel: w554 -> [w558 w562]
          tunnel: w555 -> [w559 w561]
          tunnel: w556 -> [_ w560]
          frame False {
          }
          frame True {
            n144 = case shown="True" w560 {
              selector: w560 -> [_ w569]
              tunnel: [w568 w577] -> w564
              tunnel: [w567 w576] -> w563
              tunnel: w562 -> [w565 w573]
              tunnel: w561 -> [w566 w572]
              frame False {
                n145 = call <instrlib>:"NewEraPump Stop Pump.vi"("error in (no error)"=w565, "VISA resource name"=w566) -> ("error out"=w567:errorcluster, "VISA resource name out"=w568:refnum<visa-resource-name>)  [unwired: 1 in]
              }
              frame True {
                n146 = flat-sequence {
                  tunnel: [w599] -> w575
                  tunnel: [w598] -> w574
                  tunnel: [w582] -> w570
                  tunnel: w572 -> [w595]
                  tunnel: w573 -> [w593]
                  tunnel: w569 -> [w590]
                  tunnel: w575 -> [w604]
                  tunnel: w574 -> [w603]
                  tunnel: [w602] -> w581
                  tunnel: [w601] -> w580
                  tunnel: [w600] -> w571
                  tunnel: w570 -> [w600]
                  tunnel: w581 -> [w609]
                  tunnel: w580 -> [w608]
                  tunnel: [w607] -> w579
                  tunnel: [w606] -> w578
                  tunnel: w571 -> [w605]
                  tunnel: w579 -> [w623]
                  tunnel: w578 -> [w622]
                  tunnel: [w624] -> w577
                  tunnel: [w626] -> w576
                  frame #0 {
                    w591 = 0 items=["microlitters per minute (µL/min)", "microlitters per hour (µL/hr)", "milliliters per minute (mL/min)", "milliliters per hour (µL/hr)"] ("Units")
                    w597 = u16 0 items=["Infuse", "Withdraw"] ("Direction")
                    n147 = local write "Pump #2 Purging"(w590) -> ()
                    n148 = local write "Interface Locked"(w590) -> ()
                    n149 = local read "Pump #2 Amount in Syringe (µL)"() -> (w584:dbl)
                    n150 = local read "Pump #2 flow rate (µL/min)"() -> (w589:dbl)
                    n151 = Subtract(x=w584, y="Pump #2 Partial Purge Amount (µL)") -> (x-y=w585:dbl)
                    n152 = call <instrlib>:"NE-50X Configure Rate.vi"("VISA resource name"=w595, "Flow"=w589, "Units"=w591, "error in (no error)"=w593) -> ("VISA resource name out"=w594:refnum<visa-resource-name>, "error out"=w592:errorcluster)  [unwired: 1 in]
                    n153 = Greater Or Equal?(x=w585, y=0.0) -> (x >= y?=w588:bool)
                    n154 = call <instrlib>:"NE-50X Configure Direction.vi"("error in (no error)"=w592, "Direction"=w597, "VISA resource name"=w594, "Address (0)"=0) -> ("error out"=w598:errorcluster, "VISA resource name out"=w599:refnum<visa-resource-name>)
                    n155 = Select(t=w585, s=w588, f=0.0) -> (s? t:f=w582:dbl)
                  }
                  frame #1 {
                    n156 = call <instrlib>:"NE-50X Start Pump.vi"("error in (no error)"=w603, "VISA resource name"=w604) -> ("error out"=w601:errorcluster, "VISA resource name out"=w602:refnum<visa-resource-name>)  [unwired: 1 in]
                  }
                  frame #2 {
                    n157 = while {
                      shift-right: [w614] -> w607
                      shift-left: w609 -> [w616]
                      shift-right: [w613] -> w606
                      shift-left: w608 -> [w615]
                      tunnel: w605 -> [w611]
                      stop <- w612 stop-if-true
                      n158 = call <instrlib>:"NE-50X Read Volume Dispense.vi"("VISA resource name"=w616, "error in (no error)"=w615) -> ("VISA resource name out"=w614:refnum<visa-resource-name>, "error out"=w613:errorcluster, "Amount Remaining (uL)"=w610:dbl)  [unwired: 1 in, 2 out]
                      n159 = Less Or Equal?(x=w610, y=w611) -> (x <= y?=w612:bool)
                      n160 = local write "Pump #2 Amount in Syringe (µL)"(w610) -> ()
                    }
                  }
                  frame #3 {
                    w625 = 0 items=["microlitters per minute (µL/min)", "microlitters per hour (µL/hr)", "milliliters per minute (mL/min)", "milliliters per hour (µL/hr)"] ("Units")
                    n161 = call <instrlib>:"NewEraPump Stop Pump.vi"("error in (no error)"=w622, "VISA resource name"=w623) -> ("error out"=w620:errorcluster, "VISA resource name out"=w621:refnum<visa-resource-name>)  [unwired: 1 in]
                    n162 = local read "Pump #2 flow rate (µL/min)"() -> (w619:dbl)
                    n163 = Not(x="Pump #2 Partial Purge Button") -> (.not. x?=w617:bool)
                    n164 = local write "Pump #2 Purging"(w617) -> ()
                    n165 = local write "Interface Locked"(w617) -> ()
                    n166 = call <instrlib>:"NE-50X Configure Rate.vi"("VISA resource name"=w621, "Flow"=w619, "Units"=w625, "error in (no error)"=w620) -> ("VISA resource name out"=w624:refnum<visa-resource-name>, "error out"=w626:errorcluster)  [unwired: 1 in]
                  }
                }
              }
            }
          }
        }
      }
      event "Pump #1 Full Purge Button": Value Change {
        n167 = event-data() -> ("NewVal"=w627:bool)  [unwired: 1 in, 5 out]
        n168 = local read "Pump 1 Connected"() -> (w634:bool)
        n169 = case shown="True" w634 {
          tunnel: [w636 w641] -> w631
          tunnel: [w635 w640] -> w630
          tunnel: w633 -> [w635 w639]
          tunnel: w632 -> [w636 w638]
          tunnel: w627 -> [_ w637]
          frame False {
          }
          frame True {
            n170 = case shown="True" w637 {
              selector: w637 -> [_ w646]
              tunnel: [w645 w652] -> w641
              tunnel: [w644 w651] -> w640
              tunnel: w639 -> [w642 w648]
              tunnel: w638 -> [w643 w647]
              frame False {
                n171 = call <instrlib>:"NewEraPump Stop Pump.vi"("error in (no error)"=w642, "VISA resource name"=w643) -> ("error out"=w644:errorcluster, "VISA resource name out"=w645:refnum<visa-resource-name>)  [unwired: 1 in]
              }
              frame True {
                n172 = flat-sequence {
                  tunnel: [w668] -> w650
                  tunnel: [w667] -> w649
                  tunnel: w647 -> [w664]
                  tunnel: w648 -> [w662]
                  tunnel: w646 -> [w657]
                  tunnel: w650 -> [w677]
                  tunnel: w649 -> [w676]
                  tunnel: [w675] -> w656
                  tunnel: [w674] -> w655
                  tunnel: w656 -> [w681]
                  tunnel: w655 -> [w680]
                  tunnel: [w679] -> w654
                  tunnel: [w678] -> w653
                  tunnel: w654 -> [w695]
                  tunnel: w653 -> [w693]
                  tunnel: [w696] -> w652
                  tunnel: [w698] -> w651
                  frame #0 {
                    w660 = 2 items=["microlitters per minute (µL/min)", "microlitters per hour (µL/hr)", "milliliters per minute (mL/min)", "milliliters per hour (µL/hr)"] ("Units")
                    w666 = u16 0 items=["Infuse", "Withdraw"] ("Direction")
                    n173 = local write "Interface Locked"(w657) -> ()
                    n174 = property on="Pump #1 syringe volume" class="Ring (strict)"() -> ("RingText.Text"=w659:string)  [unwired: 2 in, 2 out]
                    n175 = case shown="\"50 mL\"" w659 {
                      tunnel: [0.0 ("y") 5.0 ("y") 13.0 ("y") 14.0 ("y") 30.0 ("y")] -> w658
                      frame Default {
                      }
                      frame "5 mL" {
                      }
                      frame "15 mL" {
                      }
                      frame "20 mL" {
                      }
                      frame "50 mL" {
                      }
                    }
                    n176 = call <instrlib>:"NE-50X Configure Rate.vi"("VISA resource name"=w664, "Flow"=w658, "Units"=w660, "error in (no error)"=w662) -> ("VISA resource name out"=w663:refnum<visa-resource-name>, "error out"=w661:errorcluster)  [unwired: 1 in]
                    n177 = call <instrlib>:"NE-50X Configure Direction.vi"("error in (no error)"=w661, "Direction"=w666, "VISA resource name"=w663, "Address (0)"=0) -> ("error out"=w667:errorcluster, "VISA resource name out"=w668:refnum<visa-resource-name>)
                    "Pump #1 Purging" <- w657
                  }
                  frame #1 {
                    n178 = call <instrlib>:"NE-50X Start Pump.vi"("error in (no error)"=w676, "VISA resource name"=w677) -> ("error out"=w674:errorcluster, "VISA resource name out"=w675:refnum<visa-resource-name>)  [unwired: 1 in]
                  }
                  frame #2 {
                    n179 = while {
                      shift-right: [w686] -> w679
                      shift-left: w681 -> [w688]
                      shift-right: [w685] -> w678
                      shift-left: w680 -> [w687]
                      stop <- w682 stop-if-true
                      n180 = call <instrlib>:"NE-50X Read Volume Dispense.vi"("VISA resource name"=w688, "error in (no error)"=w687) -> ("VISA resource name out"=w686:refnum<visa-resource-name>, "error out"=w685:errorcluster, "Amount Remaining (uL)"=w684:dbl)  [unwired: 1 in, 2 out]
                      n181 = local write "Pump #1 Amount in Syringe (µL)"(w684) -> ()
                      n182 = Less Or Equal?(x=w684, y=0.0) -> (x <= y?=w682:bool)
                    }
                  }
                  frame #3 {
                    w697 = 0 items=["microlitters per minute (µL/min)", "microlitters per hour (µL/hr)", "milliliters per minute (mL/min)", "milliliters per hour (µL/hr)"] ("Units")
                    n183 = call <instrlib>:"NewEraPump Stop Pump.vi"("error in (no error)"=w693, "VISA resource name"=w695) -> ("error out"=w692:errorcluster, "VISA resource name out"=w694:refnum<visa-resource-name>)  [unwired: 1 in]
                    n184 = local read "Pump #1 flow rate (µL/min)"() -> (w691:dbl)
                    n185 = Not(x="Pump #1 Full Purge Button") -> (.not. x?=w689:bool)
                    n186 = local write "Pump #1 Purging"(w689) -> ()
                    n187 = local write "Interface Locked"(w689) -> ()
                    n188 = call <instrlib>:"NE-50X Configure Rate.vi"("VISA resource name"=w694, "Flow"=w691, "Units"=w697, "error in (no error)"=w692) -> ("VISA resource name out"=w696:refnum<visa-resource-name>, "error out"=w698:errorcluster)  [unwired: 1 in]
                  }
                }
              }
            }
          }
        }
      }
      event "Pump #2 Full Purge\n Button": Value Change {
        n189 = event-data() -> ("NewVal"=w704:bool)  [unwired: 1 in, 5 out]
        n190 = local read "Pump 2 Connected"() -> (w703:bool)
        n191 = case shown="True" w703 {
          tunnel: [w708 w713] -> w701
          tunnel: [w707 w712] -> w700
          tunnel: w705 -> [w707 w711]
          tunnel: w706 -> [w708 w710]
          tunnel: w704 -> [_ w709]
          frame False {
          }
          frame True {
            n192 = case shown="True" w709 {
              selector: w709 -> [_ w718]
              tunnel: [w717 w724] -> w713
              tunnel: [w716 w723] -> w712
              tunnel: w711 -> [w714 w720]
              tunnel: w710 -> [w715 w719]
              frame False {
                n193 = call <instrlib>:"NewEraPump Stop Pump.vi"("error in (no error)"=w714, "VISA resource name"=w715) -> ("error out"=w716:errorcluster, "VISA resource name out"=w717:refnum<visa-resource-name>)  [unwired: 1 in]
              }
              frame True {
                n194 = flat-sequence {
                  tunnel: [w740] -> w722
                  tunnel: [w739] -> w721
                  tunnel: w719 -> [w735]
                  tunnel: w720 -> [w733]
                  tunnel: w718 -> [w729]
                  tunnel: w722 -> [w749]
                  tunnel: w721 -> [w748]
                  tunnel: [w747] -> w728
                  tunnel: [w746] -> w727
                  tunnel: w728 -> [w753]
                  tunnel: w727 -> [w752]
                  tunnel: [w751] -> w726
                  tunnel: [w750] -> w725
                  tunnel: w726 -> [w767]
                  tunnel: w725 -> [w765]
                  tunnel: [w768] -> w724
                  tunnel: [w770] -> w723
                  frame #0 {
                    w736 = 2 items=["microlitters per minute (µL/min)", "microlitters per hour (µL/hr)", "milliliters per minute (mL/min)", "milliliters per hour (µL/hr)"] ("Units")
                    w738 = u16 0 items=["Infuse", "Withdraw"] ("Direction")
                    n195 = local write "Interface Locked"(w729) -> ()
                    n196 = property on="Pump #2 syringe volume" class="Ring (strict)"() -> ("RingText.Text"=w730:string)  [unwired: 2 in, 2 out]
                    n197 = case shown="\"50 mL\"" w730 {
                      tunnel: [0.0 ("y") 5.0 ("y") 13.0 ("y") 14.0 ("y") 30.0 ("y")] -> w731
                      frame Default {
                      }
                      frame "5 mL" {
                      }
                      frame "15 mL" {
                      }
                      frame "20 mL" {
                      }
                      frame "50 mL" {
                      }
                    }
                    n198 = call <instrlib>:"NE-50X Configure Rate.vi"("VISA resource name"=w735, "Flow"=w731, "Units"=w736, "error in (no error)"=w733) -> ("VISA resource name out"=w734:refnum<visa-resource-name>, "error out"=w732:errorcluster)  [unwired: 1 in]
                    n199 = call <instrlib>:"NE-50X Configure Direction.vi"("error in (no error)"=w732, "Direction"=w738, "VISA resource name"=w734, "Address (0)"=0) -> ("error out"=w739:errorcluster, "VISA resource name out"=w740:refnum<visa-resource-name>)
                    "Pump #2 Purging" <- w729
                  }
                  frame #1 {
                    n200 = call <instrlib>:"NE-50X Start Pump.vi"("error in (no error)"=w748, "VISA resource name"=w749) -> ("error out"=w746:errorcluster, "VISA resource name out"=w747:refnum<visa-resource-name>)  [unwired: 1 in]
                  }
                  frame #2 {
                    n201 = while {
                      shift-right: [w758] -> w751
                      shift-left: w753 -> [w760]
                      shift-right: [w757] -> w750
                      shift-left: w752 -> [w759]
                      stop <- w754 stop-if-true
                      n202 = call <instrlib>:"NE-50X Read Volume Dispense.vi"("VISA resource name"=w760, "error in (no error)"=w759) -> ("VISA resource name out"=w758:refnum<visa-resource-name>, "error out"=w757:errorcluster, "Amount Remaining (uL)"=w756:dbl)  [unwired: 1 in, 2 out]
                      n203 = local write "Pump #2 Amount in Syringe (µL)"(w756) -> ()
                      n204 = Less Or Equal?(x=w756, y=0.0) -> (x <= y?=w754:bool)
                    }
                  }
                  frame #3 {
                    w769 = 0 items=["microlitters per minute (µL/min)", "microlitters per hour (µL/hr)", "milliliters per minute (mL/min)", "milliliters per hour (µL/hr)"] ("Units")
                    n205 = local read "Pump #2 flow rate (µL/min)"() -> (w763:dbl)
                    n206 = Not(x="Pump #2 Full Purge\n Button") -> (.not. x?=w761:bool)
                    n207 = call <instrlib>:"NewEraPump Stop Pump.vi"("error in (no error)"=w765, "VISA resource name"=w767) -> ("error out"=w764:errorcluster, "VISA resource name out"=w766:refnum<visa-resource-name>)  [unwired: 1 in]
                    n208 = local write "Pump #2 Purging"(w761) -> ()
                    n209 = local write "Interface Locked"(w761) -> ()
                    n210 = call <instrlib>:"NE-50X Configure Rate.vi"("VISA resource name"=w766, "Flow"=w763, "Units"=w769, "error in (no error)"=w764) -> ("VISA resource name out"=w768:refnum<visa-resource-name>, "error out"=w770:errorcluster)  [unwired: 1 in]
                  }
                }
              }
            }
          }
        }
      }
    }
    n211 = local read "Pump #2 Flowing"() -> (w13:bool)
    n212 = local read "Pump #1 Flowing"() -> (w12:bool)
    n213 = case shown="True" w12 {
      tunnel: w21 -> [w54 w64]
      tunnel: w20 -> [w53 w63]
      tunnel: [w54 w56] -> w19
      tunnel: [w53 w55] -> w18
      frame False {
      }
      frame True {
        n214 = property on="Pump #1 syringe volume" class="Ring (strict)"() -> ("RingText.Text"=w62:string)  [unwired: 2 in, 2 out]
        n215 = case shown="\"50 mL\"" w62 {
          tunnel: [0.0 ("y") 5000.0 ("y") 15000.0 ("y") 20000.0 ("y") 50000.0 ("y")] -> w60
          frame Default {
          }
          frame "5 mL" {
          }
          frame "15 mL" {
          }
          frame "20 mL" {
          }
          frame "50 mL" {
          }
        }
        n216 = call <instrlib>:"NE-50X Read Volume Dispense.vi"("VISA resource name"=w64, "error in (no error)"=w63) -> ("VISA resource name out"=w57:refnum<visa-resource-name>, "error out"=w58:errorcluster, "Amount Remaining (uL)"=w61:dbl)  [unwired: 1 in, 2 out]
        n217 = Greater Or Equal?(x=w61, y=w60) -> (x >= y?=w59:bool)
        n218 = local write "Pump #1 Amount in Syringe (µL)"(w61) -> ()
        n219 = case shown="True" w59 {
          tunnel: w58 -> [w65 w71]
          tunnel: [w65 w70] -> w55
          tunnel: w57 -> [w66 w69]
          tunnel: [w66 w68] -> w56
          frame False {
          }
          frame True {
            n220 = call <instrlib>:"NewEraPump Stop Pump.vi"("error in (no error)"=w71, "VISA resource name"=w69) -> ("error out"=w70:errorcluster, "VISA resource name out"=w68:refnum<visa-resource-name>)  [unwired: 1 in]
            n221 = local write "Pump #1 Flowing"(FALSE) -> ()
          }
        }
      }
    }
    n222 = case shown="True" w13 {
      tunnel: w17 -> [w30 w40]
      tunnel: w16 -> [w29 w39]
      tunnel: [w30 w34] -> w15
      tunnel: [w29 w36] -> w14
      frame False {
      }
      frame True {
        n223 = property on="Pump #2 syringe volume" class="Ring (strict)"() -> ("RingText.Text"=w38:string)  [unwired: 2 in, 2 out]
        n224 = case shown="\"50 mL\"" w38 {
          tunnel: [0.0 ("y") 5000.0 ("y") 15000.0 ("y") 20000.0 ("y") 50000.0 ("y")] -> w33
          frame Default {
          }
          frame "5 mL" {
          }
          frame "15 mL" {
          }
          frame "20 mL" {
          }
          frame "50 mL" {
          }
        }
        n225 = call <instrlib>:"NE-50X Read Volume Dispense.vi"("VISA resource name"=w40, "error in (no error)"=w39) -> ("VISA resource name out"=w35:refnum<visa-resource-name>, "error out"=w37:errorcluster, "Amount Remaining (uL)"=w32:dbl)  [unwired: 1 in, 2 out]
        n226 = Greater Or Equal?(x=w32, y=w33) -> (x >= y?=w31:bool)
        n227 = local write "Pump #2 Amount in Syringe (µL)"(w32) -> ()
        n228 = case shown="True" w31 {
          tunnel: w37 -> [w41 w47]
          tunnel: [w41 w46] -> w36
          tunnel: w35 -> [w42 w45]
          tunnel: [w42 w44] -> w34
          frame False {
          }
          frame True {
            n229 = call <instrlib>:"NewEraPump Stop Pump.vi"("error in (no error)"=w47, "VISA resource name"=w45) -> ("error out"=w46:errorcluster, "VISA resource name out"=w44:refnum<visa-resource-name>)  [unwired: 1 in]
            n230 = local write "Pump #2 Flowing"(FALSE) -> ()
          }
        }
      }
    }
    n231 = local read "Pump 1 Connected"() -> (w22:bool)
    n232 = local read "Pump 2 Connected"() -> (w23:bool)
  }
  n233 = local write "Pump #2 Partial Purge Amount (µL)"(w2) -> ()
  n234 = property on="Pump #2 Start/Stop Button" class="Bool"("BoolText.Text"=w10) -> ()  [unwired: 2 in, 2 out]
  n235 = property on="Pump #1 Start/Stop Button" class="Bool"("BoolText.Text"=w10) -> ()  [unwired: 2 in, 2 out]
  n236 = invoke class="VI" method="Default Vals.Reinit All"(reference=w3) -> ()  [unwired: 2 in, 3 out]
  n237 = case shown="True" w4 {
    tunnel: w7 -> [_ w772]
    tunnel: w6 -> [_ w771]
    frame False {
    }
    frame True {
      w775 = T2 1 items=["no dialog", "OK message", "continue or stop message", "OK message + warnings", "continue/stop + warnings"] ("type of dialog (OK msg:1)")
      n238 = call <instrlib>:"NewEraPump Stop Pump.vi"("error in (no error)"=w771, "VISA resource name"=w772) -> ("error out"=w774:errorcluster, "VISA resource name out"=w773:refnum<visa-resource-name>)  [unwired: 1 in]
      n239 = call <instrlib>:"NE-50X Query Status.vi"("error in (no error)"=w774, "VISA resource name"=w773) -> ("error out"=w778:errorcluster, "VISA resource name out"=w779:refnum<visa-resource-name>)  [unwired: 1 in, 1 out]
      n240 = call <instrlib>:"NE-50X Reset Pump.vi"("error in (no error)"=w778, "VISA resource name"=w779) -> ("error out"=w777:errorcluster, "VISA resource name out"=w780:refnum<visa-resource-name>)
      n241 = call <instrlib>:"NE-50X Close.vi"("VISA resource name"=w780, "error in (no error)"=w777) -> ("error out"=w776:errorcluster)  [unwired: 13 in]
      n242 = call <vilib>:"General Error Handler.vi"("type of dialog (OK msg:1)"=w775, "error in (no error)"=w776) -> ()  [unwired: 9 in, 5 out]
    }
  }
  n243 = case shown="True" w5 {
    tunnel: w9 -> [_ w782]
    tunnel: w8 -> [_ w781]
    frame False {
    }
    frame True {
      n244 = call <instrlib>:"NewEraPump Stop Pump.vi"("error in (no error)"=w781, "VISA resource name"=w782) -> ("error out"=w783:errorcluster, "VISA resource name out"=w784:refnum<visa-resource-name>)  [unwired: 1 in]
      n245 = call <instrlib>:"NE-50X Query Status.vi"("error in (no error)"=w783, "VISA resource name"=w784) -> ("error out"=w786:errorcluster, "VISA resource name out"=w787:refnum<visa-resource-name>)  [unwired: 1 in, 1 out]
      n246 = call <instrlib>:"NE-50X Reset Pump.vi"("error in (no error)"=w786, "VISA resource name"=w787) -> ("error out"=w785:errorcluster, "VISA resource name out"=w788:refnum<visa-resource-name>)
      n247 = call <instrlib>:"NE-50X Close.vi"("VISA resource name"=w788, "error in (no error)"=w785) -> ()  [unwired: 13 in, 1 out]
    }
  }
  "Pump #2 Flowing" <- w1
  "Pump #1 Flowing" <- w1
  "Pump #1 Sucked Amount (µL)" <- w2
  "Pump #1 Amount in Syringe (µL)" <- w2
  "Pump #2 Amount in Syringe (µL)" <- w2
  "Pump #2 Sucked Amount (µL)" <- w2
  "Interface Locked" <- w1
